vi "Store New Used Blank.vi"(6 "2DPanelBlank":refnum<class "2DPanelBlank.lvclass">, 8 "error in (no error)":errorcluster, 9 "Col":i32, 10 "Row":i32, 11 "2DArrayManager in":refnum<class "2DArrayManager.lvclass">) -> (0 "error out":errorcluster, 3 "2DArrayManager out":refnum<class "2DArrayManager.lvclass">)   [LabVIEW 2020, in "OOPanel.lvlib" / "2DArrayManager.lvclass"]
uses:
  2DArrayManager.lvclass
  2DPanelBlank/2DPanelBlank.lvclass
  C:/dev/lv20CE/relink/lv-oopanel/OOPanel/ArrayPanel/ArrayPanel.lvclass
  2DPanelBlank/State.ctl
  2DArrayManager.lvclass/2DArrayManager.ctl
  2DPanelBlank/2DPanelBlank.lvclass/2DPanelBlank.ctl
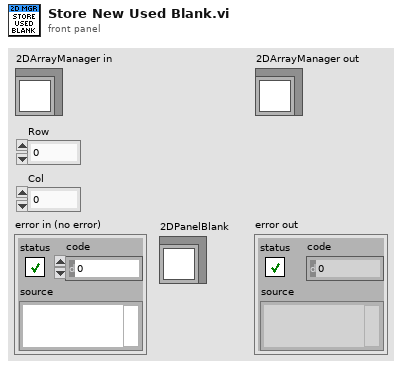
[diagram p1: front panel]
types:
  T1 = typedef "OOPanel.lvlib/2DPanelBlank.lvclass/State.ctl" = enum16{"New", "Idle", "Pool", "Used", "No SP"}
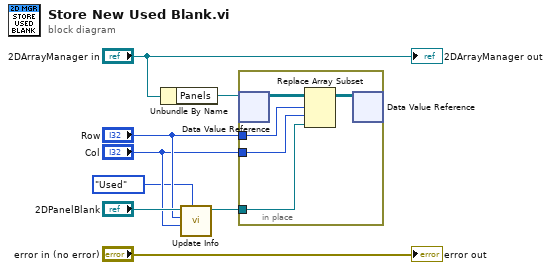
[diagram p0: block diagram]
diagram:
  n1 = Unbundle By Name("2DArrayManager in") -> ("Panels"=w7:refnum<data-value>)
  n2 = call "Update Info.vi"("State"=State."Used", "Col"="Col", "Row"="Row", "2DPanelBlank in"="2DPanelBlank") -> ("2DPanelBlank out"=w4:refnum<class "2DPanelBlank.lvclass">)  [unwired: 6 in, 1 out]
  n3 = in-place {
    in-place-border: "Row" -> [w12]
    in-place-border: "Col" -> [w11]
    in-place-border: w4 -> [w10]
    n4 = in-place-dvr #1(w7) -> (w13:refnum<class "ArrayPanel.lvclass">[][])  [unwired: 1 out]
    n5 = Replace Array Subset(array=w13, new element=w10, index (row)=w12, index (col)=w11) -> (w9:refnum<class "ArrayPanel.lvclass">[][])
    n6 = in-place-dvr #1(w9) -> ()  [unwired: 2 out]
  }
  "error out" <- "error in (no error)"
  "2DArrayManager out" <- "2DArrayManager in"
